vi "Sim_Save_CSV.vi"(10 "File Path (empty = dialog)":path, 11 "Log Records":T1[](array[typedef])) -> (2 "Saved?":bool, 3 "Status Message":string)   [LabVIEW 2019]
doc: "Writes the log records to a CSV file: one header row, then one row per record. Empty File Path opens a file dialog. The file operation is 'replace or create with confirmation', so an existing file is never overwritten silently. Numbers use a decimal point regardless of locale. Errors are reported in Status Message (43 = cancelled) and the file reference is always closed."
uses:
  Sim_Log_Record.ctl
  Sim_State_Enum.ctl
  Sim_Data.ctl
  Test_State_Enum2.ctl
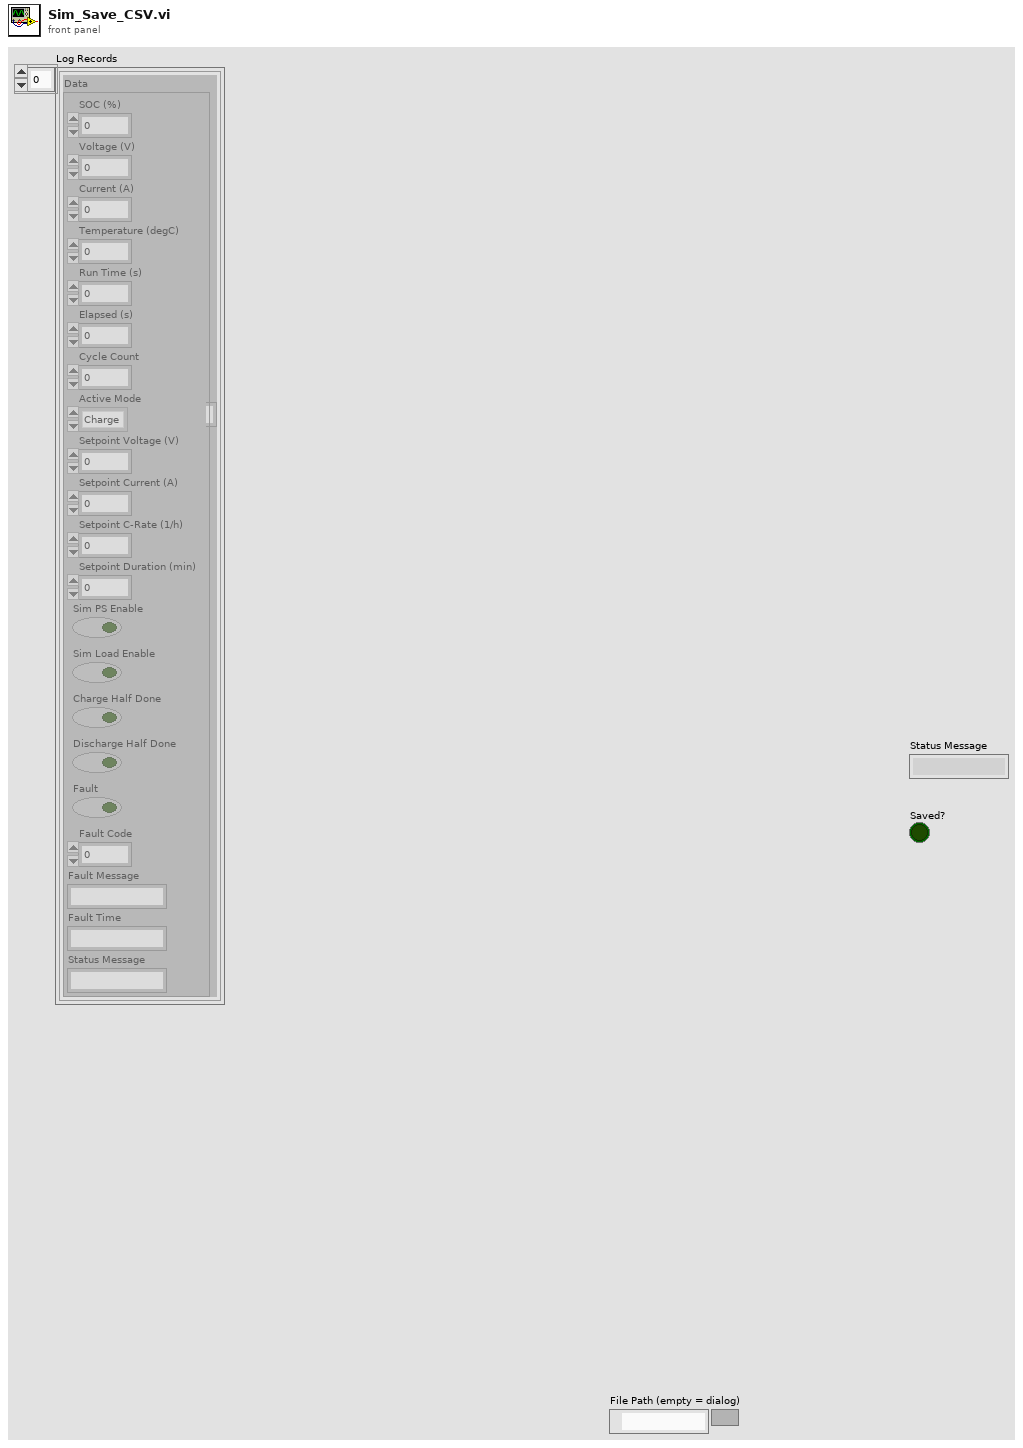
[diagram p1: front panel]
types:
  T1 = typedef "Sim_Log_Record.ctl" = cluster{"Timestamp":string, "State":T2, "Data":T3}
  T2 = typedef "Sim_State_Enum.ctl" = enum16{"INIT", "IDLE", "CHARGING", "DISCHARGING", "STOPPED", "FAULT"}
  T3 = typedef "Sim_Data.ctl" = cluster{"SOC (%)":dbl, "Voltage (V)":dbl, "Current (A)":dbl, "Temperature (degC)":dbl, "Run Time (s)":dbl, "Elapsed (s)":dbl, "Cycle Count":u32, "Active Mode":T4, "Setpoint Voltage (V)":dbl, "Setpoint Current (A)":dbl, "Setpoint C-Rate (1/h)":dbl, "Setpoint Duration (min)":dbl, "Sim PS Enable":bool, "Sim Load Enable":bool, "Charge Half Done":bool, "Discharge Half Done":bool, "Fault":bool, "Fault Code":i32, "Fault Message":string, "Fault Time":string, "Status Message":string}
  T4 = typedef "Test_State_Enum2.ctl" = enum16{"Charge", "Discharge"}
  T5 = enum16{"open", "replace", "create", "open or create", "replace or create", "replace or create with confirmation"}
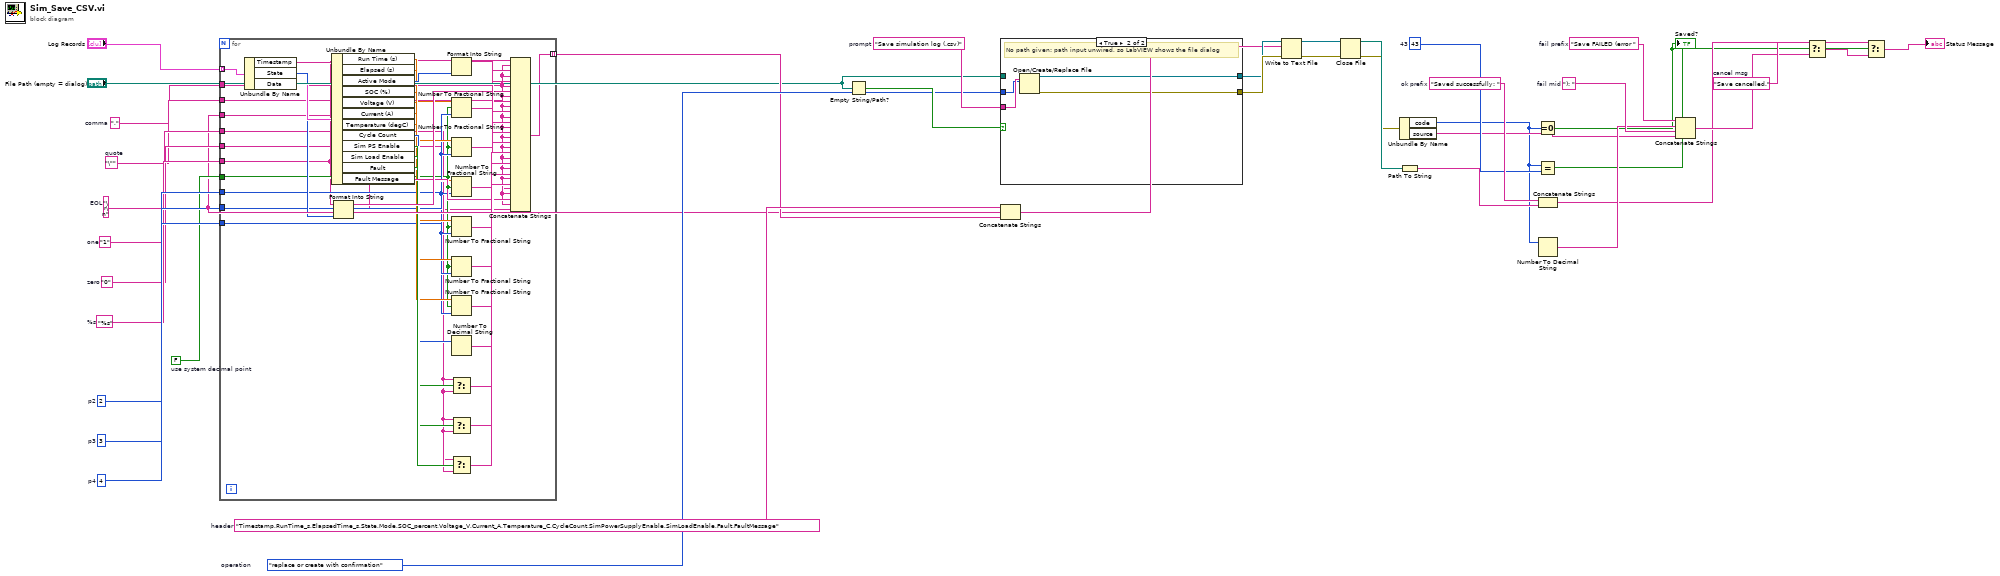
[diagram p0: block diagram]
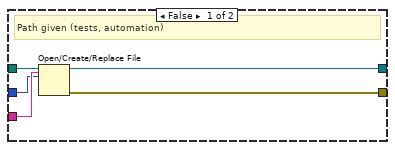
[diagram p2: hidden frame]
diagram:
  w38 = "Save cancelled."  # cancel msg
  w36 = "): "  # fail mid
  w35 = "Save FAILED (error "  # fail prefix
  w32 = "Saved successfully: "  # ok prefix
  w30 = 43  # 43
  w19 = "Save simulation log (.csv)"  # prompt
  w18 = T5."replace or create with confirmation"  # operation
  w16 = "Timestamp,RunTime_s,ElapsedTime_s,State,Mode,SOC_percent,Voltage_V,Current_A,Temperature_C,CycleCount,SimPowerSupplyEnable,SimLoadEnable,Fault,FaultMessage"  # header
  w14 = 4  # p4
  w13 = 3  # p3
  w12 = 2  # p2
  w11 = FALSE  # use system decimal point
  w10 = "%s"  # %s
  w9 = "0"  # zero
  w8 = "1"  # one
  w7 = "\r\n"  # EOL
  w6 = "\""  # quote
  w5 = ","  # comma
  n1 = for {
    tunnel: "Log Records" -> [w40] mode=indexing
    tunnel: w5 -> [w41]
    tunnel: w6 -> [w42]
    tunnel: w7 -> [w43]
    tunnel: w8 -> [w44]
    tunnel: w9 -> [w45]
    tunnel: w10 -> [w46]
    tunnel: w11 -> [w47]
    tunnel: w12 -> [w48]
    tunnel: w13 -> [w49]
    tunnel: w14 -> [w50]
    tunnel: [w78] -> w15 mode=indexing
    n2 = Unbundle By Name(w40) -> ("Timestamp"=w51:string, "State"=w52:T2, "Data"=w53:T3)
    n3 = Unbundle By Name(w53) -> ("Run Time (s)"=w54:dbl, "Elapsed (s)"=w55:dbl, "Active Mode"=w56:T4, "SOC (%)"=w57:dbl, "Voltage (V)"=w58:dbl, "Current (A)"=w59:dbl, "Temperature (degC)"=w60:dbl, "Cycle Count"=w61:u32, "Sim PS Enable"=w62:bool, "Sim Load Enable"=w63:bool, "Fault"=w64:bool, "Fault Message"=w65:string)
    n4 = Format Into String(format string=w46, w52) -> (resulting string=w66:string)  [unwired: 2 in, 1 out]
    n5 = Format Into String(format string=w46, w56) -> (resulting string=w67:string)  [unwired: 2 in, 1 out]
    n6 = Number To Fractional String(use system decimal point (T)=w47, number=w54, precision (6)=w49) -> (F-format string=w68:string)  [unwired: 1 out]
    n7 = Number To Fractional String(use system decimal point (T)=w47, number=w55, precision (6)=w49) -> (F-format string=w69:string)  [unwired: 1 out]
    n8 = Number To Fractional String(use system decimal point (T)=w47, number=w57, precision (6)=w48) -> (F-format string=w70:string)  [unwired: 1 out]
    n9 = Number To Fractional String(use system decimal point (T)=w47, number=w58, precision (6)=w50) -> (F-format string=w71:string)  [unwired: 1 out]
    n10 = Number To Fractional String(use system decimal point (T)=w47, number=w59, precision (6)=w50) -> (F-format string=w72:string)  [unwired: 1 out]
    n11 = Number To Fractional String(use system decimal point (T)=w47, number=w60, precision (6)=w48) -> (F-format string=w73:string)  [unwired: 1 out]
    n12 = Number To Decimal String(number=w61) -> (decimal integer string=w74:string)  [unwired: 1 in]
    n13 = Select(t=w44, s=w62, f=w45) -> (s? t:f=w75:string)
    n14 = Select(t=w44, s=w63, f=w45) -> (s? t:f=w76:string)
    n15 = Select(t=w44, s=w64, f=w45) -> (s? t:f=w77:string)
    n16 = Concatenate Strings(w51, w41, w68, w41, w69, w41, w66, w41, w67, w41, w70, w41, w71, w41, w72, w41, w73, w41, w74, w41, w75, w41, w76, w41, w77, w41, w42, w65, w42, w43) -> (w78:string)
  }
  n17 = Empty String/Path?(string/path="File Path (empty = dialog)") -> (empty?=w20:bool)
  n18 = case shown="True" w20 {
    tunnel: "File Path (empty = dialog)" -> [w79 _]
    tunnel: w18 -> [w80 w84]
    tunnel: w19 -> [w81 w85]
    tunnel: [w83 w87] -> w21
    tunnel: [w82 w86] -> w22
    frame False {
      # "Path given (tests, automation)"
      n19 = Open/Create/Replace File(file path (use dialog)=w79, prompt=w81, operation (0:open)=w80) -> (refnum out=w83:refnum<file>, error out=w82:errorcluster)  [unwired: 3 in, 1 out]
    }
    frame True {
      # "No path given: path input unwired, so LabVIEW shows the file dialog"
      n20 = Open/Create/Replace File(prompt=w85, operation (0:open)=w84) -> (refnum out=w87:refnum<file>, error out=w86:errorcluster)  [unwired: 4 in, 1 out]
    }
  }
  n21 = Concatenate Strings(w16, w7, w15) -> (w17:string)
  n22 = Write to Text File(file (use dialog)=w21, text=w17, error in=w22) -> (refnum out=w24:refnum<file>, error out=w23:errorcluster)  [unwired: 1 in, 1 out]
  n23 = Close File(refnum=w24, error in=w23) -> (path=w26:path, error out=w25:errorcluster)
  n24 = Unbundle By Name(w25) -> ("code"=w27:i32, "source"=w28:string)
  n25 = Path To String(path=w26) -> (string=w29:string)
  n26 = Equal To 0?(x=w27) -> (x = 0?=w4:bool)
  "Saved?" <- w4
  n27 = Equal?(x=w27, y=w30) -> (x = y?=w31:bool)
  n28 = Concatenate Strings(w32, w29) -> (w33:string)
  n29 = Number To Decimal String(number=w27) -> (decimal integer string=w34:string)  [unwired: 1 in]
  n30 = Concatenate Strings(w35, w34, w36, w28) -> (w37:string)
  n31 = Select(t=w38, s=w31, f=w37) -> (s? t:f=w39:string)
  n32 = Select(t=w33, s=w4, f=w39) -> (s? t:f=→"Status Message":string)
